vi "Get All Arguments.vi"(9 "error in (no error)":errorcluster) -> (1 "error out":errorcluster, 2 "data":string[](array[string]), 3 "arguments":string[](array[string]), 4 "arguments as text":string)   [LabVIEW 2019, in "Error Generation.lvlib"]
doc: "Get all arguments and the data.\nNo arguments founds = empty Arrays\n- - -\nCopyright (c) 2023, Merecs Engineering GmbH"
uses:
  <vilib>/regexp/Match Regular Expression.xnode
  Error Generation.lvlib
panel:
  # "Connector Pane"
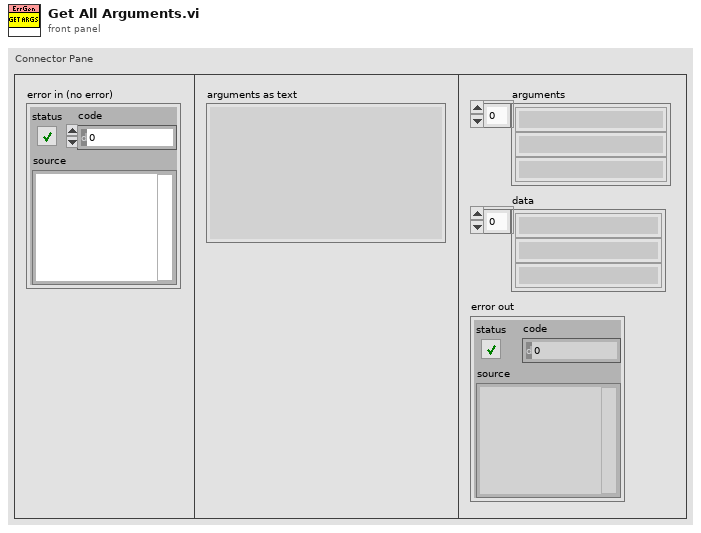
[diagram p1: front panel]
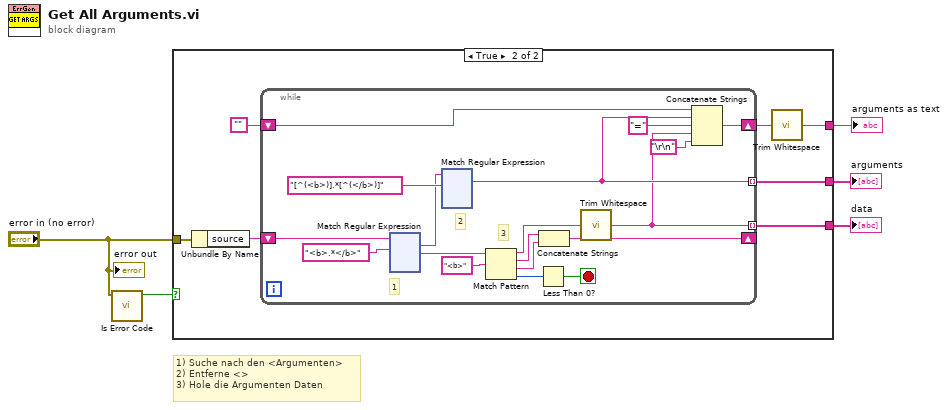
[diagram p0: block diagram]
diagram:
  # "1) Suche nach den <Argumenten>\n2) Entferne <>\n3) Hole die Argumenten Daten"
  n1 = call "Is Error Code.vi"("error in (no error)"="error in (no error)") -> ("Code!=0"=w4:bool)  [unwired: 5 in, 1 out]
  n2 = case shown="True" w4 {
    tunnel: [_ w12] -> w2
    tunnel: "error in (no error)" -> [_ w11]
    tunnel: [_ w9] -> w3
    tunnel: [_ w6] -> w1
    frame False {
    }
    frame True {
      n3 = Unbundle By Name(w11) -> ("source"=w10:string)
      n4 = while {
        tunnel: [w13] -> w12 mode=indexing
        shift-right: [w19] -> _
        shift-left: w10 -> [w26]
        tunnel: [w18] -> w9 mode=indexing
        shift-right: [w16] -> w8
        shift-left: "" -> [w15]
        stop <- w22 stop-if-true
        # "3"
        # "2"
        # "1"
        n5 = xnode "Match Regular Expression"("input string"=w26, "regular expression"="<b>.*</b>" ("format string")) -> ("whole match"=w20:string, "after match"=w27:string)  [unwired: 4 in, 3 out]
        n6 = xnode "Match Regular Expression"("input string"=w20, "regular expression"="[^(<b>)].*[^(</b>)]") -> ("whole match"=w18:string)  [unwired: 4 in, 4 out]
        n7 = Match Pattern(string=w27, regular expression="<b>") -> (before substring=w29:string, match substring=w25:string, after substring=w24:string, offset past match=w23:i32)  [unwired: 1 in]
        n8 = Less Than 0?(x=w23) -> (x < 0?=w22:bool)
        n9 = Concatenate Strings(w25, w24) -> (w19:string)
        n10 = call <vilib>:"Trim Whitespace.vi"("string"=w29) -> ("trimmed string"=w13:string)  [unwired: 1 in]
        n11 = Concatenate Strings(w15, w18, "=" ("string"), w13, "\r\n") -> (w16:string)
      }
      n12 = call <vilib>:"Trim Whitespace.vi"("string"=w8) -> ("trimmed string"=w6:string)  [unwired: 1 in]
    }
  }
  "arguments" <- w3
  "data" <- w2
  "arguments as text" <- w1
  "error out" <- "error in (no error)"
